vi "Add Array Items To Schema.vi"(8 "error in":errorcluster, 10 "input parameter":T1, 11 "schema":string) -> (0 "error out":errorcluster, 3 "schema out":string)   [LabVIEW 2020, in "MCP Server.lvlib"]
doc: "Completes the JSON schema of one tool input. sub type of the input holds the JSON Schema of its LabVIEW type, made by LV Type To JSON Schema.vi: items for arrays of any dimension (an element type without a JSON equivalent gives \"items\":{}), properties for clusters, format date-time for timestamps and the item names of enums. It is merged into the input's schema (type, description), so its members are added and its type wins. An input whose sub type is empty is passed through unchanged. Finally an empty description is left out of the schema (Remove Empty Description.vi): it tells a client nothing."
uses:
  MCP Server.lvlib
  <vilib>/JDP Science/JSONtext/Get all Object Items.vi
  <vilib>/JDP Science/JSONtext/Set Multiple Object Items.vi
  <vilib>/JDP Science/JSONtext/JSONtext.lvlib
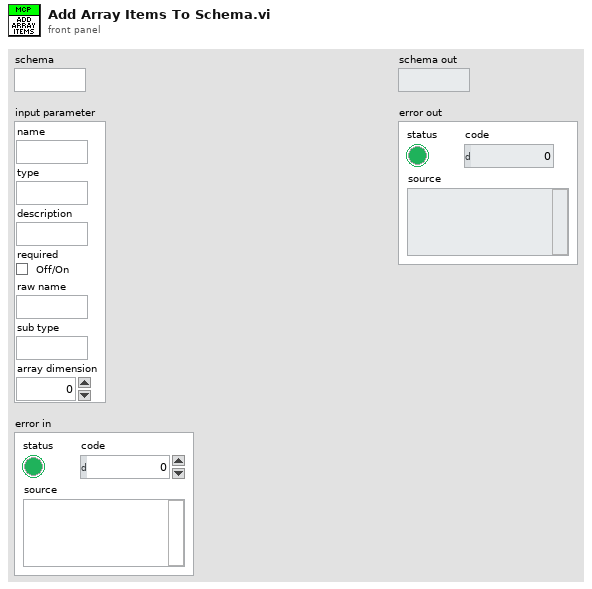
[diagram p1: front panel]
types:
  T1 = cluster{"name":string, "type":string, "description":string, "required":bool, "raw name":string, "sub type":string, "array dimension":i32}
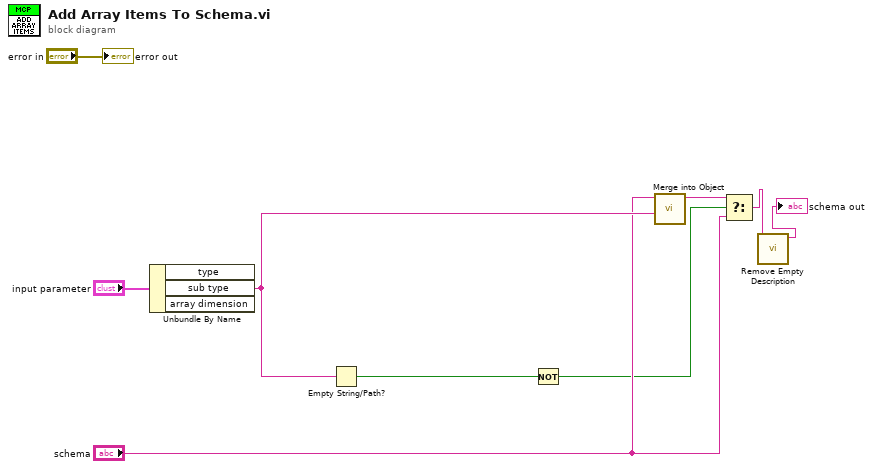
[diagram p0: block diagram]
diagram:
  n1 = Unbundle By Name("input parameter") -> ("sub type"=w6:string)  [unwired: 2 out]
  n2 = Empty String/Path?(string/path=w6) -> (empty?=w8:bool)
  n3 = Not(x=w8) -> (.not. x?=w3:bool)
  n4 = call <vilib>:"Merge into Object.vi"("JSON Object to Merge"=w6, "JSON"="schema") -> ("<JSON>"=w4:string)  [unwired: 7 in, 1 out]
  n5 = Select(t=w4, s=w3, f="schema") -> (s? t:f=w2:string)
  n6 = call "Remove Empty Description.vi"("schema"=w2) -> ("schema out"=→"schema out":string)  [unwired: 10 in]
  "error out" <- "error in"
